vi "LinearSystemId_IdentifyPositionSystem.vi"(10 "kA":dbl, 11 "kV":dbl) -> (0 "Size Coerced":bool, 3 "Linearsystem":T1)   [LabVIEW 2019, in "Trajectory_Library.lvlib"]
doc: "Identify a position system from it's kV (volts/(unit/sec)) and kA (volts/(unit/sec^2). These constants cam be found using frc-characterization. The states of the system are [position, velocity]?, inputs are [voltage], and outputs are [position].\n\nThe distance unit you choose MUST be an SI unit (i.e. meters or radians). You can use the Util.Units subVI for converting between unit types.\n \nInputs:\n - kV -- The velocity gain, in volts per (units per second)\n - kA -- The acceleration gain, in volts per (units per second squared)\n\nOutputs:\n - LinearSystem -- A LinearSystem representing the given characterized constants.\n - SizeCoerced -- A value of TRUE indicates an unexpected error occured.\n\nAdditional information:\n See https://github.com/wpilibsuite/frc-characterization @SuppressWarnings(\"ParameterName\")"
uses:
  Trajectory_Library.lvlib
  TypeDef/LINEAR_SYSTEM.ctl
  <vilib>/Analysis/Matrix/Datatypes/RealMatrix.ctl
  <vilib>/Analysis/Matrix/NI_Matrix.lvlib
panel:
  # "<States,States>"
  # "<States,Inputs>"
  # "<Outputs,States>"
  # "<Outputs,Inputs>"
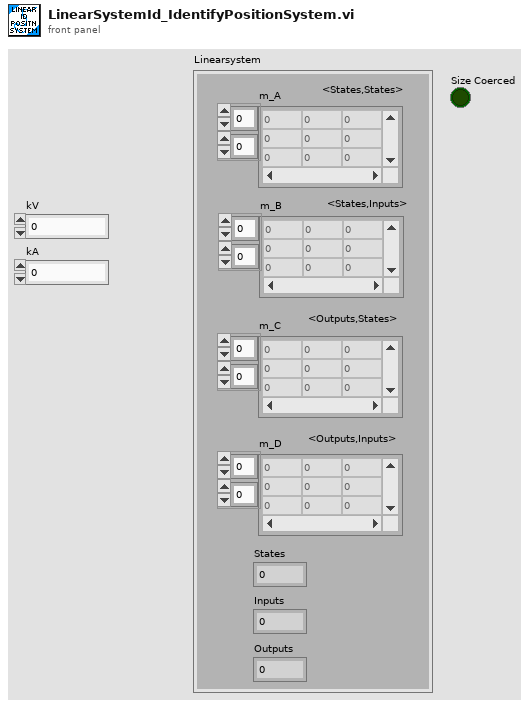
[diagram p1: front panel]
types:
  T1 = typedef "Trajectory_Library.lvlib/LINEAR_SYSTEM.ctl" = cluster{"m_A":T2, "m_B":T2, "m_C":T2, "m_D":T2, "States":i32, "Inputs":i32, "Outputs":i32}
  T2 = typedef "NI_Matrix.lvlib/RealMatrix.ctl" = dbl[][]
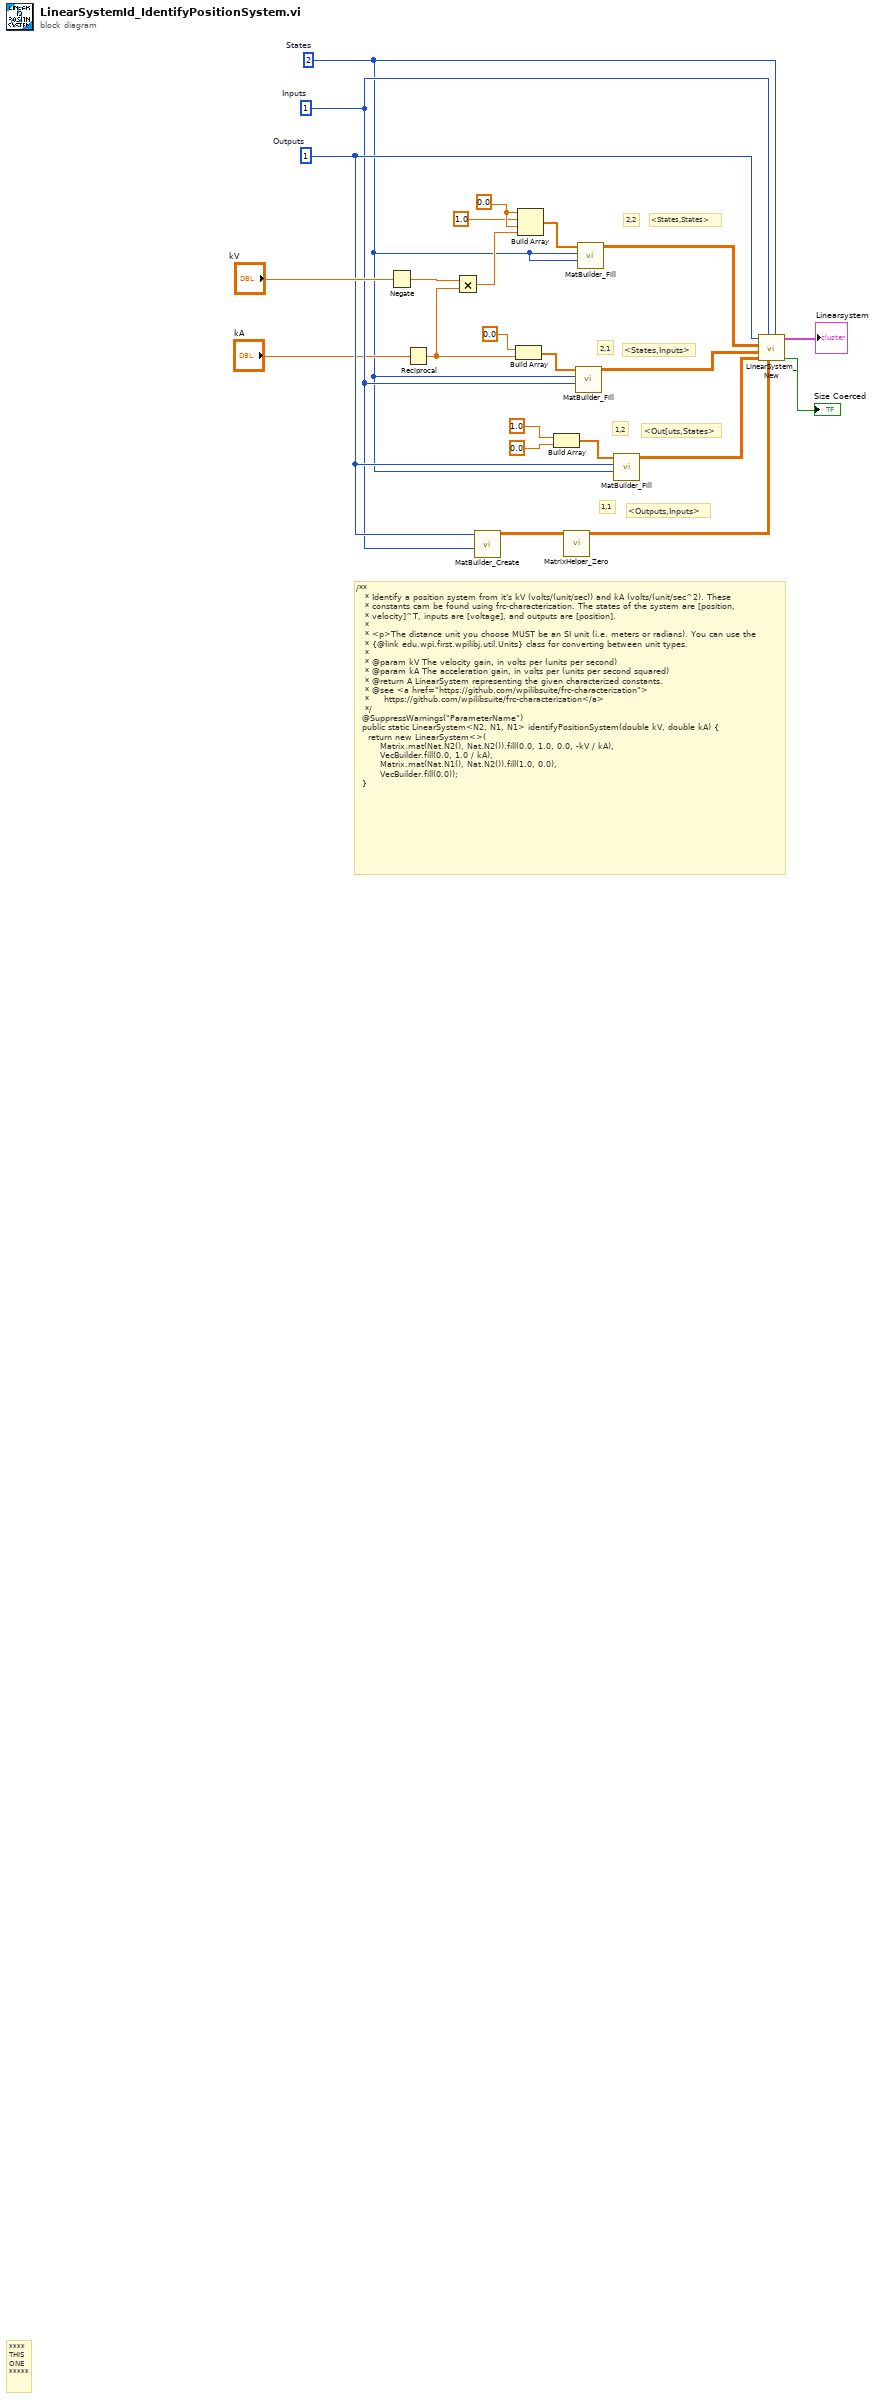
[diagram p0: block diagram]
diagram:
  w19 = 1  # Outputs
  w14 = 1  # Inputs
  w3 = 2  # States
  w6 = 0.0 ("new element/submatrix")
  # "2,2"
  # "2,1"
  # "1,2"
  # "1,1"
  # "<States,States>"
  # "<States,Inputs>"
  # "<Out[uts,States>"
  # "<Outputs,Inputs>"
  # "/**\n   * Identify a position system from it's kV (volts/(unit/sec)) and kA (volts/(unit/sec^2). These\n   * constants cam be found using frc-characterization. The states of the system are [position,\n   * velocity]^T, inputs are [voltage], and outputs are [position].\n   *\n   * <p>The distance unit you choose MUST be an SI unit (i.e. meters or radians). You can use the\n   * {@link edu.wpi.first.wpilibj.util.Units} class for converting between unit types.\n   *\n   * @param kV The velocity gain, in volts per (units per second)\n   * @param kA The acceleration gain, in volts per (units per second squared)\n   * @return A LinearSystem representing the given characterized constants.\n   * @see <a href=\"https://github.com/wpilibsuite/frc-characterization\">\n   *     https://github.com/wpilibsuite/frc-characterization</a>\n   */\n  @SuppressWarnings(\"ParameterName\")\n  public static LinearSystem<N2, N1, N1> identifyPositionSystem(double kV, double kA) {\n    return new LinearSystem<>(\n        Matrix.mat(Nat.N2(), Nat.N2()).fill(0.0, 1.0, 0.0, -kV / kA),\n        VecBuilder.fill(0.0, 1.0 / kA),\n        Matrix.mat(Nat.N1(), Nat.N2()).fill(1.0, 0.0),\n        VecBuilder.fill(0.0));\n  }"
  # "****\nTHIS\nONE\n*****"
  n1 = Negate(x="kV") -> (-x=w9:dbl)
  n2 = Reciprocal(x="kA") -> (1/x=w8:dbl)
  n3 = Multiply(x=w9, y=w8) -> (x*y=w4:dbl)
  n4 = call "MatBuilder_Create.vi"("Columns"=w14, "Rows"=w19) -> ("output matrix"=w21:T2)  [unwired: 9 in]
  n5 = Build Array(0.0 ("element"), w8) -> (w13:dbl[])
  n6 = Build Array(w6, 1.0 ("element"), w6, w4) -> (w7:dbl[])
  n7 = Build Array(1.0 ("new element/submatrix"), 0.0 ("new element/submatrix")) -> (w16:dbl[])
  n8 = call "MatrixHelper_Zero.vi"("input matrix"=w21) -> ("output matrix"=w20:T2)  [unwired: 10 in]
  n9 = call "MatBuilder_Fill.vi"("Columns"=w14, "Rows"=w3, "Value List"=w13) -> ("output matrix"=w10:T2)  [unwired: 8 in]
  n10 = call "MatBuilder_Fill.vi"("Columns"=w3, "Rows"=w3, "Value List"=w7) -> ("output matrix"=w2:T2)  [unwired: 8 in]
  n11 = call "MatBuilder_Fill.vi"("Columns"=w3, "Rows"=w19, "Value List"=w16) -> ("output matrix"=w15:T2)  [unwired: 8 in]
  n12 = call "LinearSystem_New.vi"("States"=w3, "D"=w20, "Inputs"=w14, "C"=w15, "B"=w10, "A"=w2, "Outputs"=w19) -> ("Size Coerced"=→"Size Coerced":bool, "Linearsystem"=→"Linearsystem":T1)  [unwired: 3 in]
